vi "New Channel--Dialog.vi"(8 "error in (no error)":errorcluster, 10 "Channels":string[](array[string]), 11 "ChannelManagerUI in":refnum<class "ChannelManagerUI.lvclass">) -> (0 "error out":errorcluster, 1 "OK":bool, 2 "Class":refnum<class "Channel.lvclass">, 3 "ChannelManagerUI out":refnum<class "ChannelManagerUI.lvclass">)   [LabVIEW 2021, in "Channel.lvlib" / "ChannelManagerUI.lvlib" / "ChannelManagerUI.lvclass"]
uses:
  ChannelManagerUI.lvclass
  Channel_class/Channel.lvclass
  ChannelManagerUI.lvclass/ChannelManagerUI.ctl
  Channel.lvlib
panel:
  out "Valid?":bool
  in  "Channel Name":string
  in  "OK Button":bool
  in  "Cancel Button":bool
  in  "Specific Channel":string(combo)
  in  "Channel Type":string(combo)
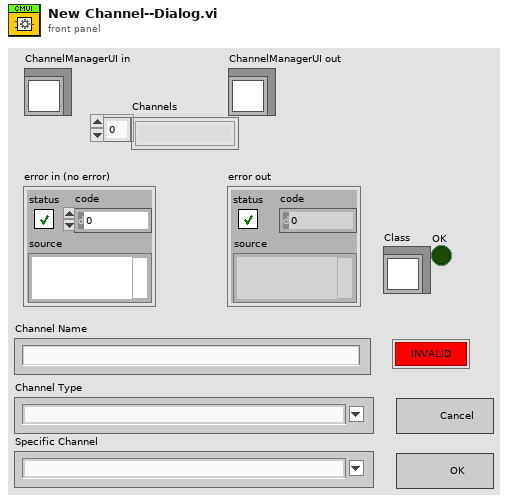
[diagram p1: front panel]
types:
  T1 = enum8{"Enabled", "Disabled", "Disabled and Grayed Out"}
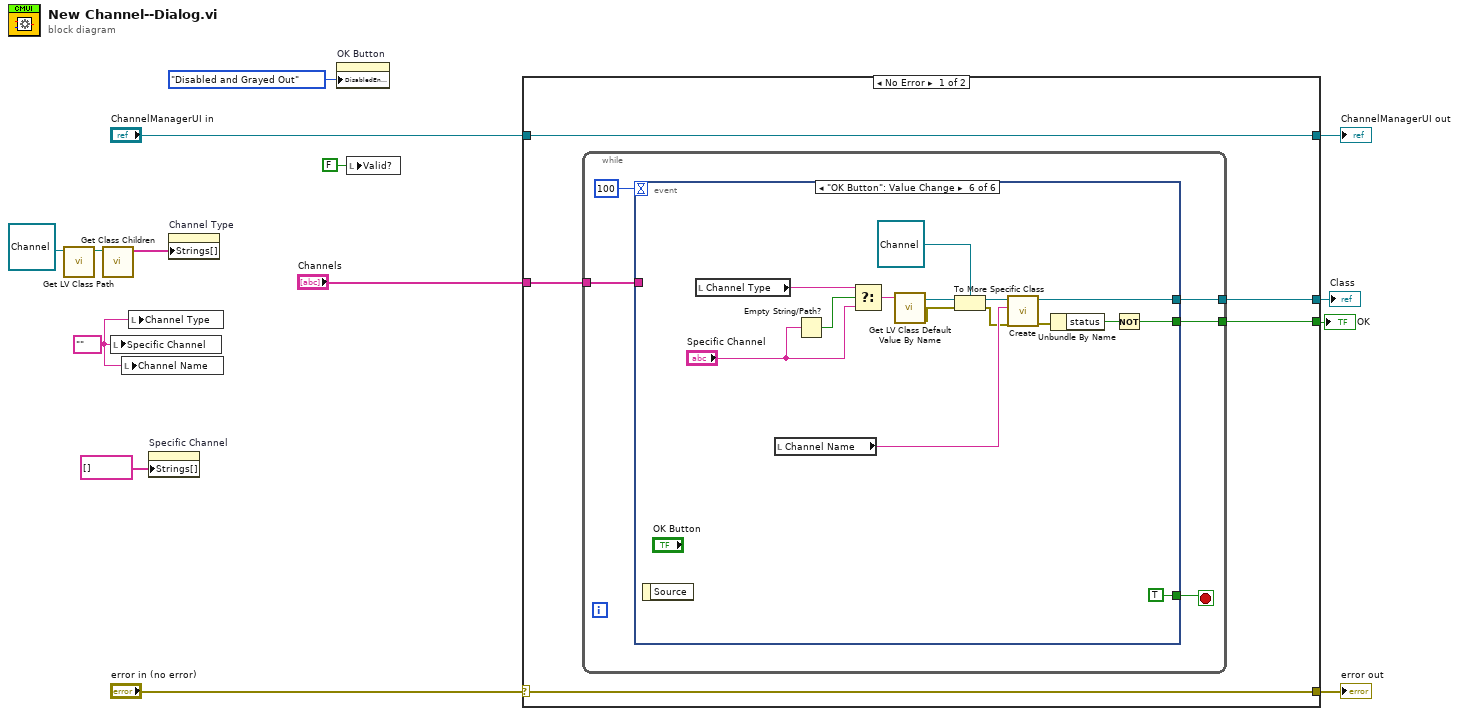
[diagram p0: block diagram]
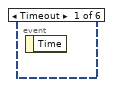
[diagram p2: hidden frame]
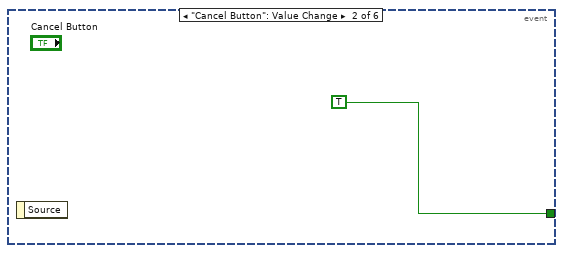
[diagram p3: hidden frame]
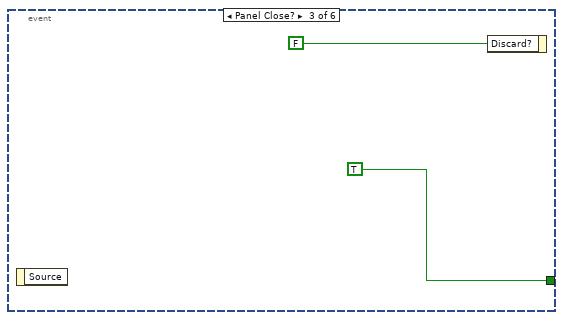
[diagram p4: hidden frame]
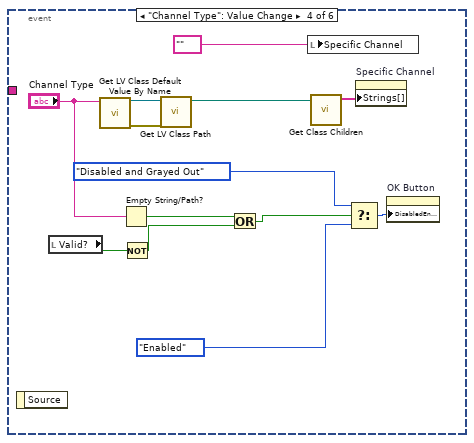
[diagram p5: hidden frame]
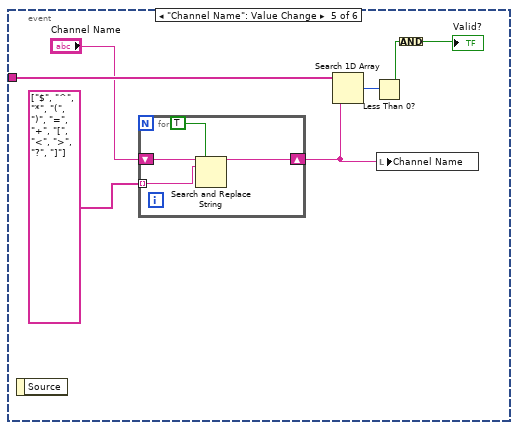
[diagram p6: hidden frame]
diagram:
  w5 = "" ("Specific Channel")
  n1 = call <vilib>:"Get LV Class Path.vi"("object"=refnum<class "Channel.lvclass"> refnum ("Channel.lvlib:Channel")) -> ("class path"=w9:path)  [unwired: 9 in, 1 out]
  n2 = call "Get Class Children.vi"("LV Class Path"=w9) -> ("Names"=w8:string[])  [unwired: 8 in, 2 out]
  n3 = local write "Specific Channel"(w5) -> ()
  n4 = local write "Channel Name"(w5) -> ()
  n5 = local write "Channel Type"(w5) -> ()
  n6 = property on="Specific Channel" class="CmbBox"("Strings[]"=string[] [] ("Strings []")) -> ()  [unwired: 2 in, 2 out]
  n7 = property on="Channel Type" class="CmbBox"("Strings[]"=w8) -> ()  [unwired: 2 in, 2 out]
  n8 = property on="OK Button" class="Bool"("DisabledEnum"=T1."Disabled and Grayed Out" ("Disabled")) -> ()  [unwired: 2 in, 2 out]
  n9 = local write "Valid?"(FALSE ("Valid?")) -> ()
  n10 = case shown="No Error" "error in (no error)" {
    selector: "error in (no error)" -> [w18 w68]
    tunnel: [w18 w68] -> w13
    tunnel: [w19 w67] -> w11
    tunnel: "ChannelManagerUI in" -> [w19 w67]
    tunnel: "Channels" -> [w17 _]
    tunnel: [w16 _] -> w2
    tunnel: [w15 _] -> w1
    frame No Error {
      n11 = while {
        tunnel: w17 -> [w22]
        tunnel: [w21] -> w16
        tunnel: [w20] -> w15
        stop <- w23 stop-if-true
        n12 = event shown="[5] \"OK Button\": Value Change" {
          selector: _ -> [_ _ _ _ _ _]
          dyn-events: _ -> [_ _ _ _ _ _]
          timeout: 100 -> [_ _ _ _ _ _]
          tunnel: [_ TRUE TRUE _ _ TRUE] -> w23
          tunnel: w22 -> [_ _ _ _ w47 _]
          tunnel: [_ _ _ _ _ w54] -> w21
          tunnel: [_ _ _ _ _ w53] -> w20
          event Timeout {
            n13 = event-data() -> ()  [unwired: 1 in, 1 out]
          }
          event "Cancel Button": Value Change {
            n14 = event-data() -> ()  [unwired: 1 in, 1 out]
          }
          event Panel Close? {
            n15 = event-data() -> ()  [unwired: 1 in, 1 out]
            n16 = event-data("Discard?"=FALSE) -> ()  [unwired: 1 in, 1 out]
          }
          event "Channel Type": Value Change {
            n17 = event-data() -> ()  [unwired: 1 in, 1 out]
            n18 = local read "Valid?"() -> (w30:bool)
            n19 = call <vilib>:"Get LV Class Default Value By Name.vi"("class name"="Channel Type") -> ("error out"=w39:errorcluster, "object"=w40:refnum<class>)  [unwired: 9 in]
            n20 = Empty String/Path?(string/path="Channel Type") -> (empty?=w32:bool)
            n21 = Not(x=w30) -> (.not. x?=w28:bool)
            n22 = call <vilib>:"Get LV Class Path.vi"("error in (no error)"=w39, "object"=w40) -> ("class path"=w38:path)  [unwired: 8 in, 1 out]
            n23 = Or(x=w32, y=w28) -> (x .or. y?=w29:bool)
            n24 = local write "Specific Channel"("" ("Specific Channel")) -> ()
            n25 = call "Get Class Children.vi"("LV Class Path"=w38) -> ("Names"=w37:string[])  [unwired: 8 in, 2 out]
            n26 = Select(t=T1."Disabled and Grayed Out" ("Disabled"), s=w29, f=T1."Enabled") -> (s? t:f=w34:T1)
            n27 = property on="Specific Channel" class="CmbBox"("Strings[]"=w37) -> ()  [unwired: 2 in, 2 out]
            n28 = property on="OK Button" class="Bool"("DisabledEnum"=w34) -> ()  [unwired: 2 in, 2 out]
          }
          event "Channel Name": Value Change {
            n29 = event-data() -> ()  [unwired: 1 in, 1 out]
            n30 = for {
              shift-right: [w50] -> w41
              shift-left: "Channel Name" -> [w51]
              tunnel: string[] ["$", "^", "*", "(", ")", "=", "+", "[", "<", ">", "?", "]"] -> [w48] mode=indexing
              n31 = Search and Replace String(replace all?=TRUE ("replace all? (F)"), input string=w51, search string=w48) -> (result string=w50:string)  [unwired: 5 in, 3 out]
            }
            n32 = Search 1D Array(1D array=w47, element=w41) -> (index of element=w45:i32)  [unwired: 1 in]
            n33 = Less Than 0?(x=w45) -> (x < 0?=w44:bool)
            n34 = local write "Channel Name"(w41) -> ()
            n35 = Compound Arithmetic op=AND(w44) -> (→"Valid?":bool)
          }
          event "OK Button": Value Change {
            n36 = event-data() -> ()  [unwired: 1 in, 1 out]
            n37 = local read "Channel Type"() -> (w66:string)
            n38 = local read "Channel Name"() -> (w59:string)
            n39 = Empty String/Path?(string/path="Specific Channel") -> (empty?=w65:bool)
            n40 = Select(t=w66, s=w65, f="Specific Channel") -> (s? t:f=w64:string)
            n41 = call <vilib>:"Get LV Class Default Value By Name.vi"("class name"=w64) -> ("error out"=w58:errorcluster, "object"=w62:refnum<class>)  [unwired: 9 in]
            n42 = To More Specific Class(target class=refnum<class "Channel.lvclass"> refnum ("Channel.lvlib:Channel"), reference=w62, error in=w58) -> (specific class reference=w60:refnum<class "Channel.lvclass">, error out=w57:errorcluster)
            n43 = call-dynamic "Create.vi"("error in (no error)"=w57, "Name"=w59, "object in"=w60) -> ("error out"=w56:errorcluster, "object out"=w54:refnum<class "Channel.lvclass">)  [unwired: 7 in]
            n44 = Unbundle By Name(w56) -> ("status"=w55:bool)
            n45 = Not(x=w55) -> (.not. x?=w53:bool)
          }
        }
      }
    }
    frame Error {
    }
  }
  "error out" <- w13
  "ChannelManagerUI out" <- w11
  "Class" <- w2
  "OK" <- w1
